vi "FuncVI-HistX.vi"(5 "InstanceRef":T2, 9 "arg list":T1[](array[typedef]) {"num" format="%.2f"}) -> (0 "error out":bool, 3 "result":T1 {"num" format="%.2f"})   [LabVIEW 2021]
doc: "::: CalcExpress Toolkit :::\nCopyright (c) 2000-2026 Konstantin Shifershteyn. All rights reserved."
uses:
  cetypes.llb/CalcExpress Function Argument Info.ctl
  cetypes.llb/CalcExpress Instance RefNum.ctl
  <vilib>/Analysis/NI_AALBase.lvlib
panel:
  in  "max arg num":i32=2
  in  "min arg num":i32=1
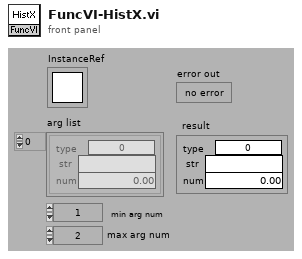
[diagram p1: front panel]
types:
  T1 = typedef "CalcExpress Function Argument Info.ctl" = cluster{"type":u32, "str":string, "num":dbl}
  T2 = typedef "CalcExpress Instance RefNum.ctl" = refnum<k1>
  T3 = enum32{"String", "DBL Number", "identifier", "1D Array of DBL", "2D Array of DBL", "CDB Number", "1D Array of CDB", "2D Array of CDB", "1D Array of String", "2D Array of String", "Unknown data type"}
  T4 = cluster{"use this constant to specify a predefined type":enum32{"String", "DBL Number", "identifier", "1D Array of DBL", "2D Array of DBL", "CDB Number", "1D Array of CDB", "2D Array of CDB", "1D Array of String", "2D Array of String", "Unknown data type"}, "data string":string, dbl}
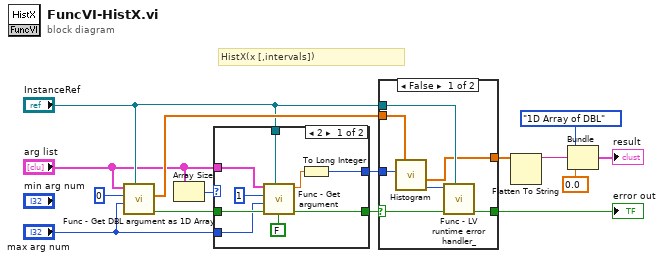
[diagram p0: block diagram]
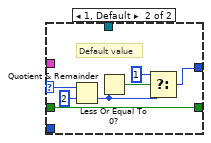
[diagram p2: hidden frame]
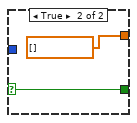
[diagram p3: hidden frame]
diagram:
  # "HistX(x [,intervals])"
  n1 = call "Func - Get DBL argument as 1D Array.vi"("InstanceRef"="InstanceRef", "max arg num"="max arg num", "arg idx"=0, "arg list"="arg list") -> ("error out"=w10:bool, "1D data"=w15:dbl[])  [unwired: 4 in, 2 out]
  n2 = Array Size(array="arg list") -> (size(s)=w6:i32)
  n3 = case shown="2" w6 {
    selector: w6 -> [_ w30]
    tunnel: w10 -> [w24 w31]
    tunnel: [w23 w31] -> w9
    tunnel: "InstanceRef" -> [w22 _]
    tunnel: "max arg num" -> [w20 _]
    tunnel: "arg list" -> [w18 _]
    tunnel: [w16 w25] -> w7
    frame 2 {
      n4 = call "Func - Get argument.vi"("ena NonNum? (F)"=FALSE, "InstanceRef"=w22, "error in"=w24, "max arg num"=w20, "arg idx"=1, "arg list"=w18) -> ("error out"=w23:bool, "num"=w17:dbl)  [unwired: 2 out]
      n5 = To Long Integer(number=w17) -> (32bit integer=w16:i32)
    }
    frame 1, Default {
      # "Default value"
      n6 = Quotient & Remainder(x=w30, y=2) -> (floor(x/y)=w28:i32)  [unwired: 1 out]
      n7 = Less Or Equal To 0?(x=w28) -> (x <= 0?=w27:bool)
      n8 = Select(t=1, s=w27, f=w28) -> (s? t:f=w25:i32)
    }
  }
  n9 = case shown="False" w9 {
    selector: w9 -> [w38 w40]
    tunnel: w15 -> [w34 _]
    tunnel: [w37 w40] -> w13
    tunnel: "InstanceRef" -> [w36 _]
    tunnel: w7 -> [w33 _]
    tunnel: [w32 dbl[] [] ("X Values")] -> w4
    frame False {
      n10 = call <vilib>:"Histogram.vi"("intervals"=w33, "X"=w34) -> ("error"=w35:i32, "X Values"=w32:dbl[])  [unwired: 6 in, 2 out]
      n11 = call "Func - LV runtime error handler_.vi"("InstanceRef"=w36, "error in"=w38, "LabVIEW error code"=w35) -> ("error out"=w37:bool)  [unwired: 8 in]
    }
    frame True {
    }
  }
  "error out" <- w13
  n12 = Flatten To String(anything=w4) -> (data string=w3:string)  [unwired: 3 in, 2 out]
  n13 = Bundle("use this constant to specify a predefined type"=T3."1D Array of DBL", "data string"=w3, 0.0) -> (→"result":T4)  [unwired: 1 in]
